vi "get_value_for_string.vi"(8 "error in (no error)":errorcluster, 11 "Value in":refnum<class "Value.lvclass">) -> (0 "error out":errorcluster, 3 "string_value":string)   [LabVIEW 2020, in "toml_edit.lvlib" / "Value.lvclass"]
uses:
  Value.lvclass
  value_type--enum.ctl
  Value.lvclass/Value.ctl
  toml_edit.lvlib
  dragon_toml_64.dll
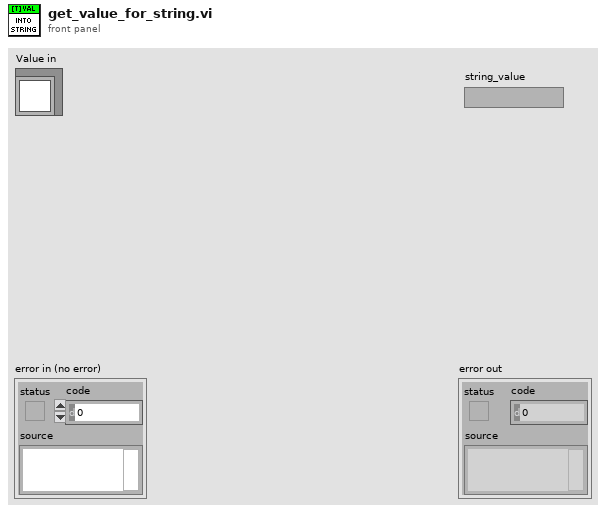
[diagram p1: front panel]
types:
  T1 = typedef "toml_edit.lvlib/Value.lvclass/value_type--enum.ctl" = enum16{"Unknown", "String", "Integer", "Float", "Boolean", "Datetime", "Array", "InlineTable"}
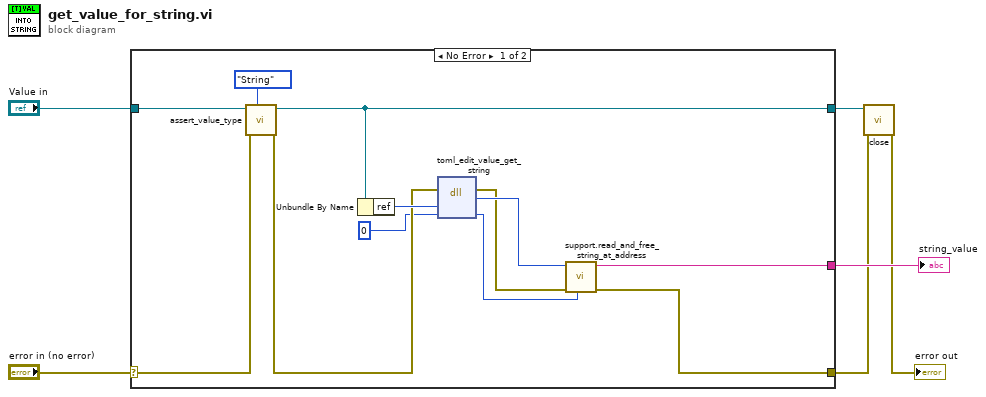
[diagram p0: block diagram]
diagram:
  n1 = case shown="No Error" "error in (no error)" {
    selector: "error in (no error)" -> [w12 w19]
    tunnel: "Value in" -> [w13 w20]
    tunnel: [w15 _] -> w4
    tunnel: [w10 w19] -> w3
    tunnel: [w9 w20] -> w2
    frame No Error {
      n2 = call "assert_value_type.vi"("value_type"=value_type--enum."String", "error in (no error)"=w12, "Value in"=w13) -> ("error out"=w11:errorcluster, "Value out"=w9:refnum<class "Value.lvclass">)  [unwired: 7 in]
      n3 = Unbundle By Name(w9) -> ("ref"=w16:u64)
      n4 = dll-call lib="C:/projects/dragon-desktop/source/submodules/toml-edit-labview/lv_src/dragon_toml_*.*" fn="toml_edit_value_get_string"(error in=w11, "item_ref"=w16, "num_bytes"=u32 0) -> (error out=w17:errorcluster, "string_ptr"=w18:u64, "num_bytes"=w7:u32)  [unwired: 3 in, 1 out]
      n5 = call "support.read_and_free_string_at_address.vi"("string_length"=w7, "error in (no error)"=w17, "string_ptr"=w18) -> ("error out"=w10:errorcluster, "string"=w15:string)  [unwired: 7 in]
    }
    frame Error {
    }
  }
  "string_value" <- w4
  n6 = call "close.vi"("error in (no error)"=w3, "Value in"=w2) -> ("error out"=→"error out":errorcluster)  [unwired: 9 in]
